vi "Func - get function name_.vi"() -> (0 "found":bool, 2 "FuncVI name":string, 3 "Func name":string)   [LabVIEW 2021]
doc: "This VI returns the name of the FuncVI and the name of its function when it is called within a FuncVI hierarchy. Refer to the VI help for more details.\n\n::: CalcExpress Toolkit :::\nCopyright (c) 2000-2026 Konstantin Shifershteyn. All rights reserved."
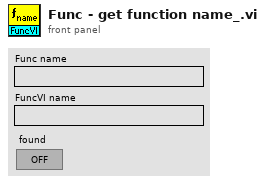
[diagram p1: front panel]
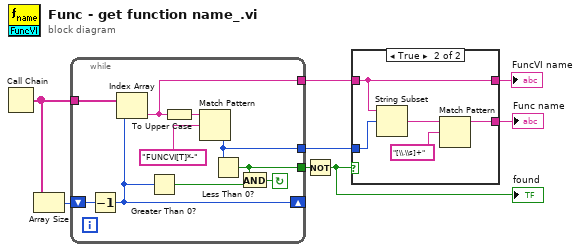
[diagram p0: block diagram]
diagram:
  n1 = Call Chain() -> (call chain=w5:string[])
  n2 = Array Size(array=w5) -> (size(s)=w1:i32)
  n3 = while {
    tunnel: [w14] -> w8
    tunnel: [w11] -> w7
    tunnel: [w16] -> w6
    tunnel: w5 -> [w12]
    shift-right: [w9] -> _
    shift-left: w1 -> [w13]
    stop <- w18 continue-if-true
    n4 = Decrement(x=w13) -> (x-1=w9:i32)
    n5 = Index Array(array=w12, index=w9) -> (element=w11:string)
    n6 = Greater Than 0?(x=w9) -> (x > 0?=w10:bool)
    n7 = To Upper Case(1:w11) -> (0:w15:string)
    n8 = Match Pattern(string=w15, regular expression="FUNCVI[T]*-") -> (offset past match=w14:i32)  [unwired: 1 in, 3 out]
    n9 = Less Than 0?(x=w14) -> (x < 0?=w16:bool)
    n10 = And(x=w16, y=w10) -> (x .and. y?=w18:bool)
  }
  n11 = Not(x=w6) -> (.not. x?=w4:bool)
  "found" <- w4
  n12 = case shown="True" w4 {
    tunnel: [_ w20] -> w3
    tunnel: [_ w23] -> w2
    tunnel: w7 -> [_ w23]
    tunnel: w8 -> [_ w22]
    frame False {
    }
    frame True {
      n13 = String Subset(string=w23, offset (0)=w22) -> (substring=w21:string)  [unwired: 1 in]
      n14 = Match Pattern(string=w21, regular expression="[\\.\\s]+") -> (before substring=w20:string)  [unwired: 1 in, 3 out]
    }
  }
  "Func name" <- w3
  "FuncVI name" <- w2
